vi "Get Supported Boolean Tables.vi"(1 "Input?":bool) -> (0 "Supported Tables":T1[](array[typedef]))   [LabVIEW 2026, in "Modbus.lvlib" / "Modbus.lvclass"]
uses:
  Modbus.lvclass
  Types/Modbus Table.ctl
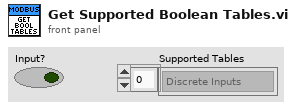
[diagram p1: front panel]
types:
  T1 = typedef "Modbus.lvlib/Modbus.lvclass/Modbus Table.ctl" = enum16{"Discrete Inputs", "Coils", "Input Registers", "Holding Registers"}
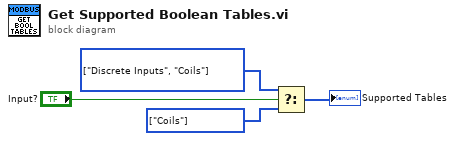
[diagram p0: block diagram]
diagram:
  w2 = T1[] [enum."Coils"] items=["Discrete Inputs", "Coils", "Input Registers", "Holding Registers"]
  w1 = T1[] [enum."Discrete Inputs", enum."Coils"] items=["Discrete Inputs", "Coils", "Input Registers", "Holding Registers"]
  n1 = Select(t=w1, s="Input?", f=w2) -> (s? t:f=→"Supported Tables":T1[])
